vi "Anal tzt close header_MS.vi"(6 "A TDMS refnum":refnum<k34>, 8 "error in":errorcluster caption="エラー入力", 9 "B Table refnum":refnum<file>, 10 "R Table refnum":refnum<file>, 11 "S Table refnum":refnum<file>) -> (0 "error out":errorcluster caption="エラー出力")   [LabVIEW 2018]
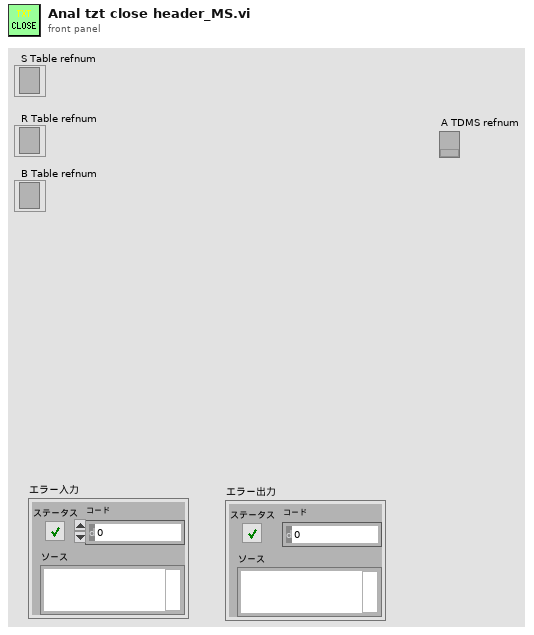
[diagram p1: front panel]
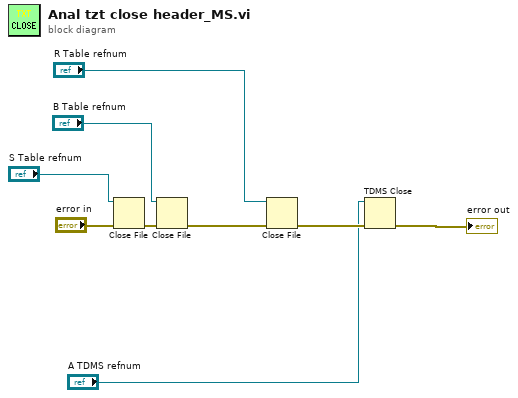
[diagram p0: block diagram]
diagram:
  n1 = Close File(refnum="S Table refnum", error in="error in") -> (error out=w7:errorcluster)  [unwired: 1 out]
  n2 = Close File(refnum="B Table refnum", error in=w7) -> (error out=w2:errorcluster)  [unwired: 1 out]
  n3 = Close File(refnum="R Table refnum", error in=w2) -> (error out=w5:errorcluster)  [unwired: 1 out]
  n4 = TDMS Close(8:w5, 11:"A TDMS refnum") -> (0:→"error out":errorcluster)  [unwired: 1 out]
